vi "Solar_Tracking_System.vi"() -> ()   [LabVIEW 2025]
panel:
  out "LDR 2 Value":dbl
  out "LDR 1 Value":dbl
  out "LDR2":bool
  out "LDR 2":u8(slide) scale=0.0..100.0
  out "LDR 1":u8(slide) scale=0.0..100.0
  out "LDR1":bool
  out "Diraction of the light":dbl(knob) scale=0.0..10.0
  in  "VISA Resource Name":refnum<visa-resource-name>
  in  "Stop Button":bool
  in  "Byte Count":u32
  # "Solar Tracking System"
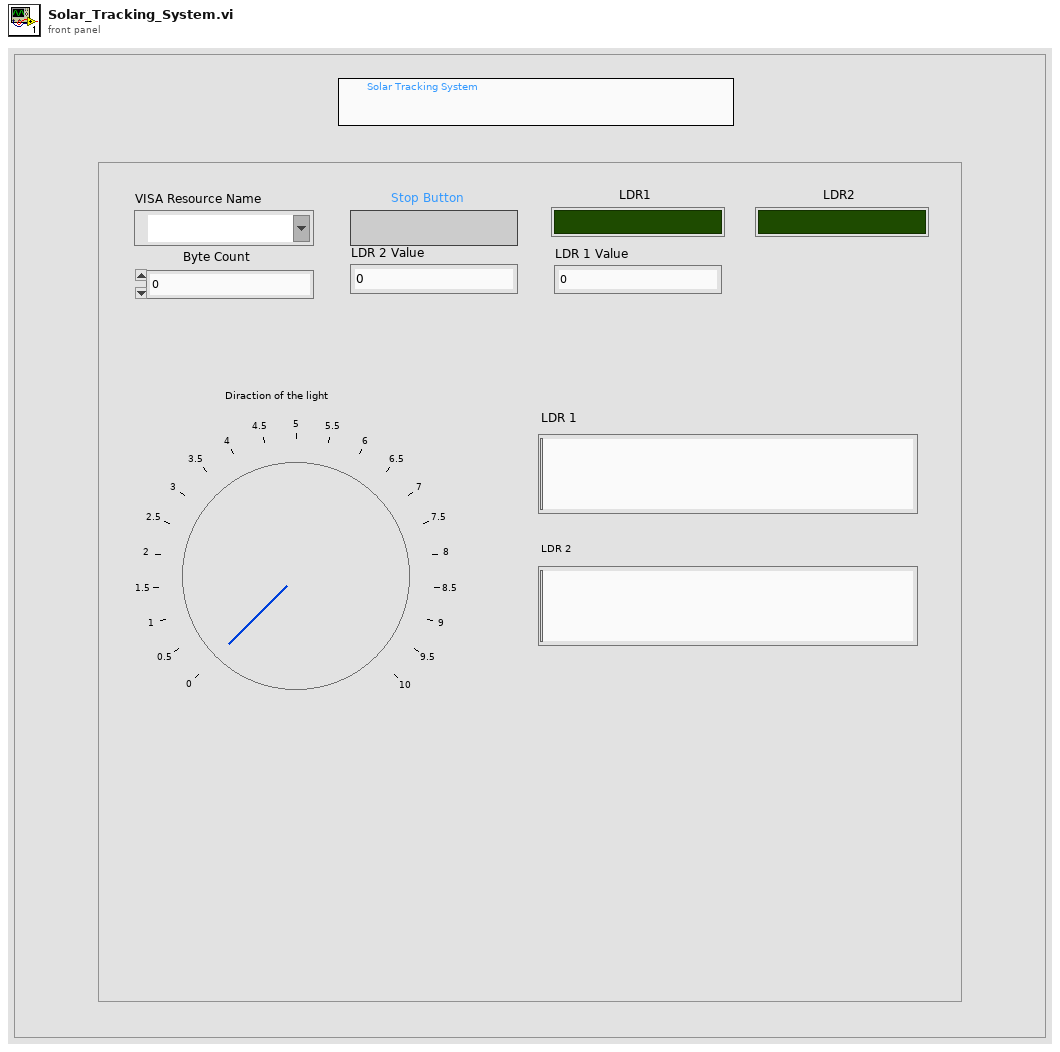
[diagram p1: front panel]
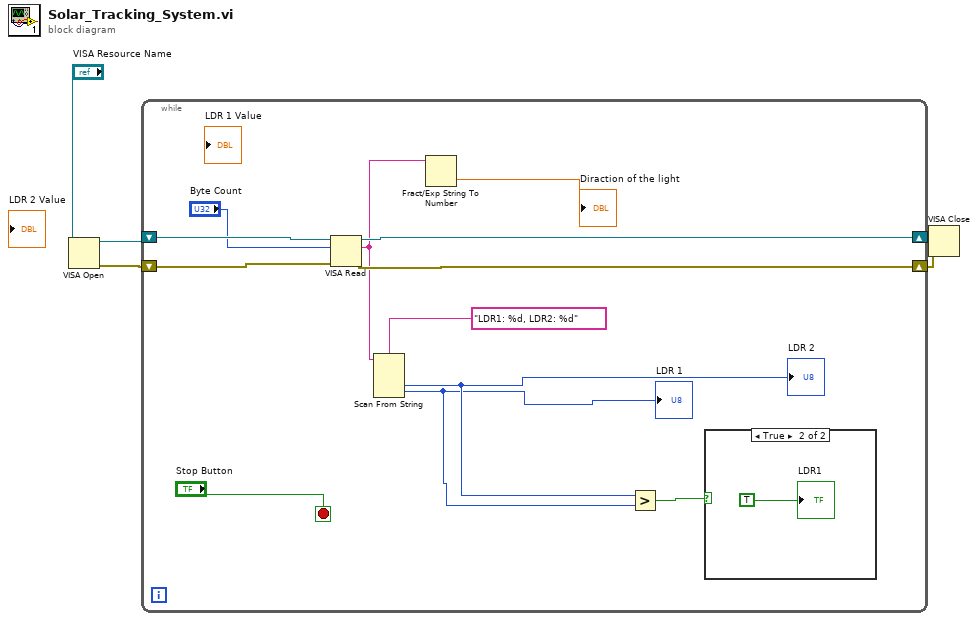
[diagram p0: block diagram]
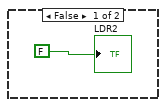
[diagram p2: hidden frame]
diagram:
  n1 = VISA Open(VISA resource name="VISA Resource Name") -> (VISA resource name=w3:refnum<visa-resource-name>, error out=w5:errorcluster)  [unwired: 4 in]
  n2 = while {
    shift-right: [w14] -> w2
    shift-left: w3 -> [w15]
    shift-right: [w16] -> w4
    shift-left: w5 -> [w17]
    stop <- "Stop Button" stop-if-true
    n3 = VISA Read(VISA resource name=w15, byte count="Byte Count", error in (no error)=w17) -> (VISA resource name out=w14:refnum<visa-resource-name>, read buffer=w10:string, error out=w16:errorcluster)  [unwired: 1 out]
    n4 = Scan From String "Scan From String"(format string="LDR1: %d, LDR2: %d", input string=w10) -> (output 1=w8:u8, output 2=w7:u8)  [unwired: 4 in, 3 out]
    "LDR 1" <- w7
    "LDR 2" <- w8
    n5 = Fract/Exp String To Number(string=w10) -> (number=→"Diraction of the light":dbl)  [unwired: 3 in, 1 out]
    n6 = Greater?(x=w8, y=w7) -> (0:w6:bool)
    n7 = case shown="True" w6 {
      frame False {
        "LDR2" <- FALSE ("Boolean")
      }
      frame True {
        "LDR1" <- TRUE
      }
    }
  }
  n8 = VISA Close(VISA resource name=w2, error in (no error)=w4) -> ()  [unwired: 1 out]
